vi "upload.start_part_upload.vi"(6 "Part Number":i32, 8 "error in":errorcluster, 10 "File Part Binary":string, 11 "Multipart Upload":refnum<class "Multipart Upload.lvclass">) -> (0 "error out":errorcluster, 3 "Multipart Upload out":refnum<class "Multipart Upload.lvclass">)   [LabVIEW 2020, in "Multipart Upload.lvclass"]
uses:
  Multipart Upload.lvclass
  Multipart Upload.lvclass/Multipart Upload.ctl
  upload.part_core.vi
  Nominal Client/Nominal Client.lvclass
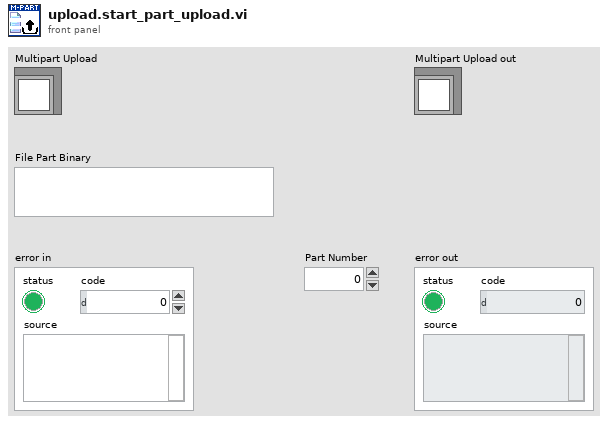
[diagram p1: front panel]
types:
  T1 = map{i32, cluster{"url":string, "headers":map{string, string}}}
  T2 = cluster{"url":string, "headers":map{string, string}}
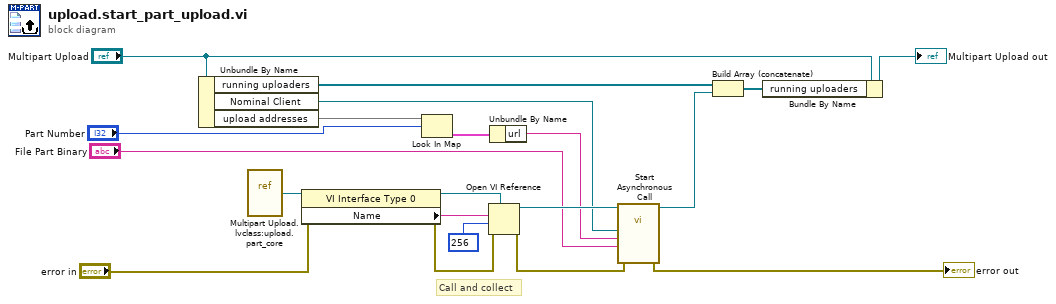
[diagram p0: block diagram]
diagram:
  # "Call and collect"
  n1 = Unbundle By Name("Multipart Upload") -> ("running uploaders"=w10:refnum<vi>[], "Nominal Client"=w2:refnum<class "Nominal Client.lvclass">, "upload addresses"=w6:T1)
  n2 = vi-ref "Multipart Upload.lvclass:upload.part_core.vi"() -> (w16:refnum<vi>)
  n3 = property class="VI Interface Type 0"(reference=w16, error in="error in") -> (reference out=w14:refnum<vi>, error out=w12:errorcluster, "Name"=w15:string)
  n4 = Look In Map(map=w6, key="Part Number") -> (value=w4:T2)  [unwired: 1 in, 1 out]
  n5 = Open VI Reference(type specifier VI Refnum (for type only)=w14, vi path=w15, options=256, error in (no error)=w12) -> (vi reference=w19:refnum<vi>, error out=w18:errorcluster)  [unwired: 2 in]
  n6 = Unbundle By Name(w4) -> ("url"=w3:string)
  n7 = call-by-ref "Start Asynchronous Call"(reference=w19, error in=w18, "Body"="File Part Binary", "Full Path"=w3, "Nominal Client"=w2) -> (reference out=w9:refnum<vi>, error out=→"error out":errorcluster)  [unwired: 7 in, 2 out]
  n8 = Build Array (concatenate)(w10, w9) -> (w1:refnum<vi>[])
  n9 = Bundle By Name(cluster="Multipart Upload", "running uploaders"=w1) -> (→"Multipart Upload out":refnum<class "Multipart Upload.lvclass">)
